vi "Scripting_ReplaceVisAndControls.vi"(0 "ViRef":refnum<vi>, 1 "OldVIsAndControls":path[](array[path]), 2 "NewVIsAndControls":path[](array[path]), 5 "error in (no error)":errorcluster) -> (15 "ReplacedVIsConPaneSize":u32[](array[numeric]), 19 "error out":errorcluster)   [LabVIEW 2020]
uses:
  <resource>/Framework/Providers/Open_GDS/ClassProviders/Common/ScriptingFunctions/Scripting.lvclass
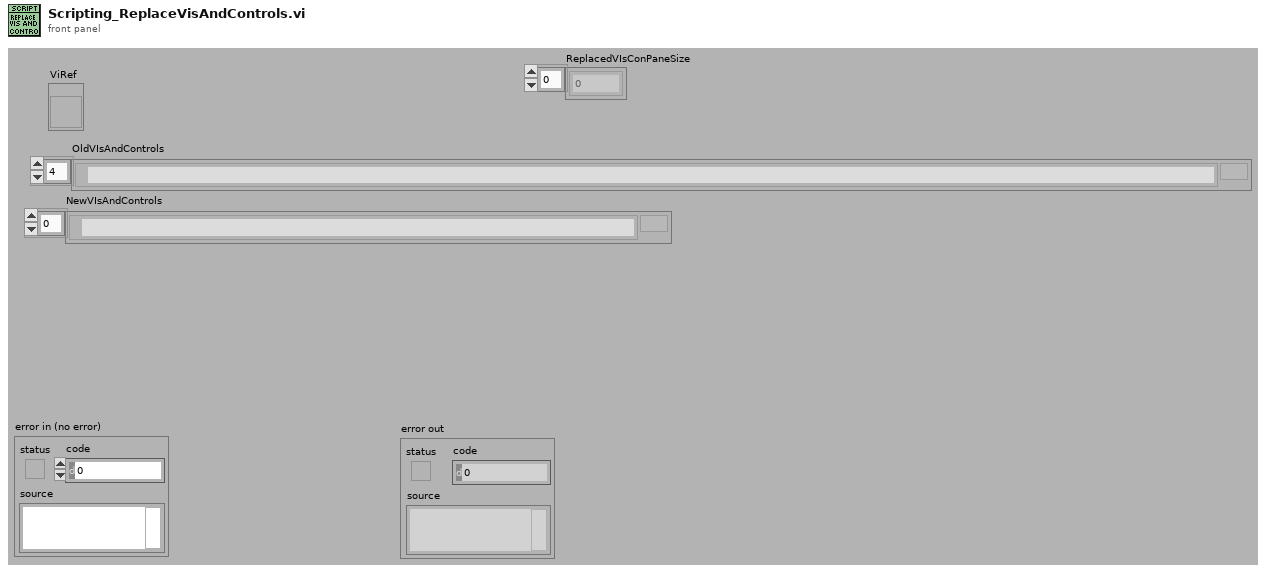
[diagram p1: front panel]
types:
  T1 = enum32{"invalid lock state", "Not Locked", "Locked (No Password)", "Password-protected"}
  T2 = cluster{"ClassControls":refnum<vi>[], "NewClassControl":path, "ReplacedVIsConPaneSize":u32[]}
  T3 = enum32{"not a typedef", "typedef", "strict typedef", "class private data"}
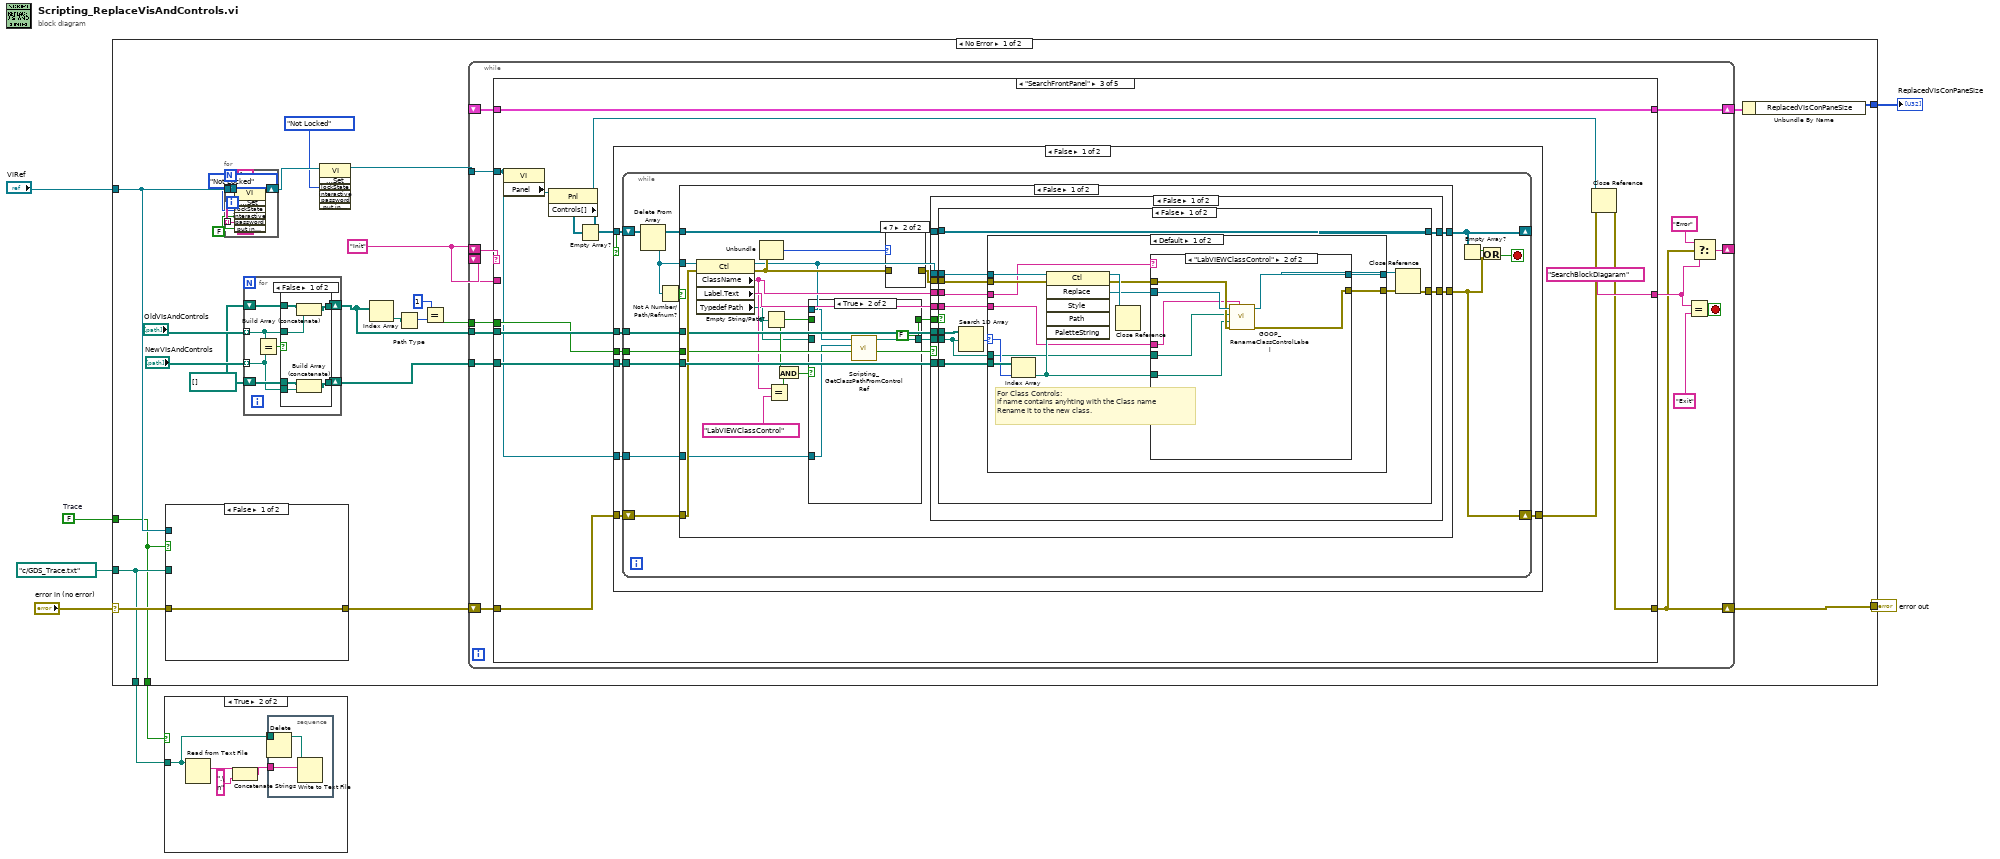
[diagram p0: block diagram]
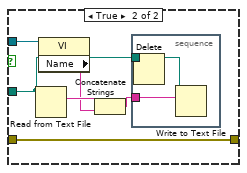
[diagram p3: hidden frame]
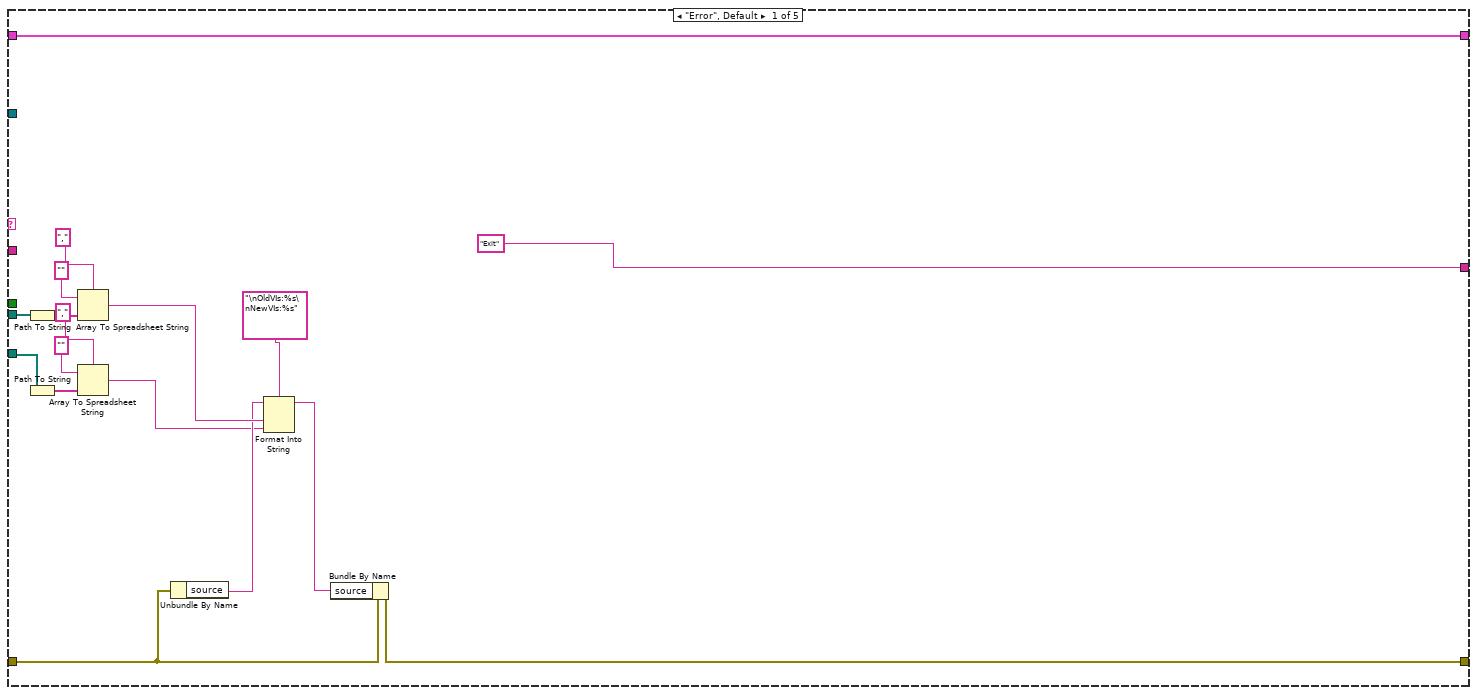
[diagram p5: hidden frame]
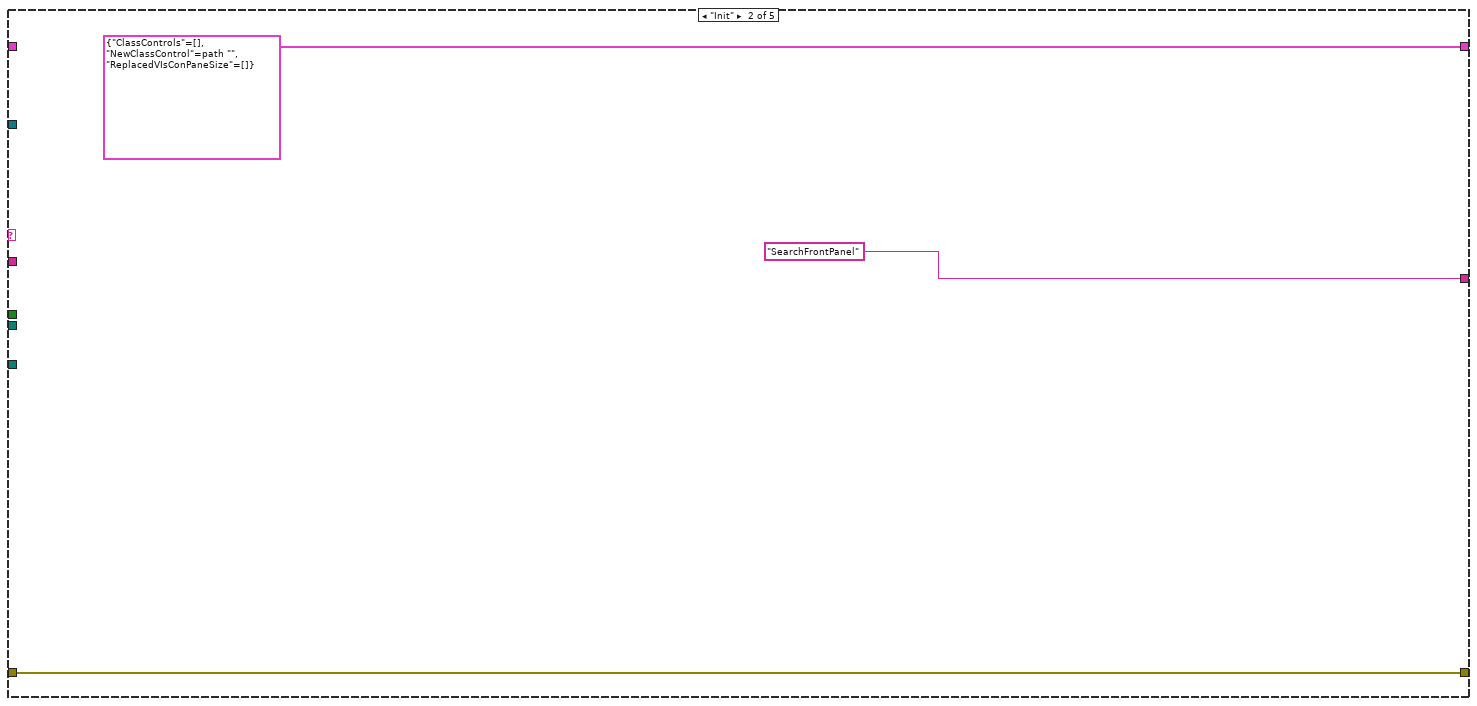
[diagram p6: hidden frame]
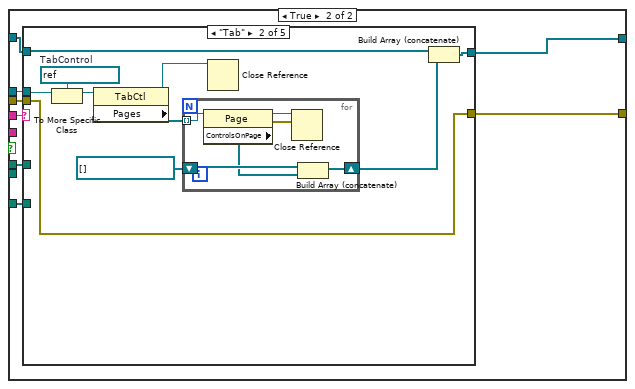
[diagram p11: hidden frame]
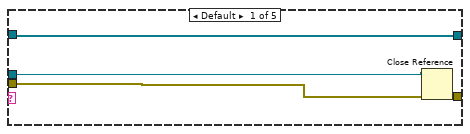
[diagram p12: hidden frame]
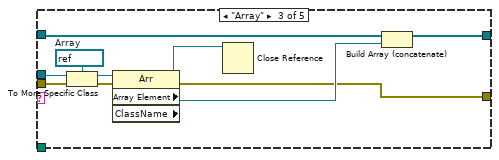
[diagram p13: hidden frame]
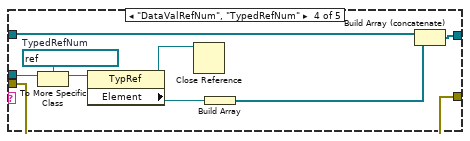
[diagram p14: hidden frame]
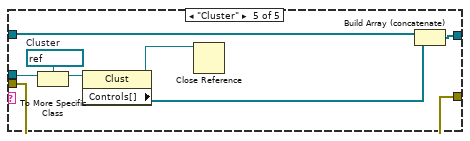
[diagram p15: hidden frame]
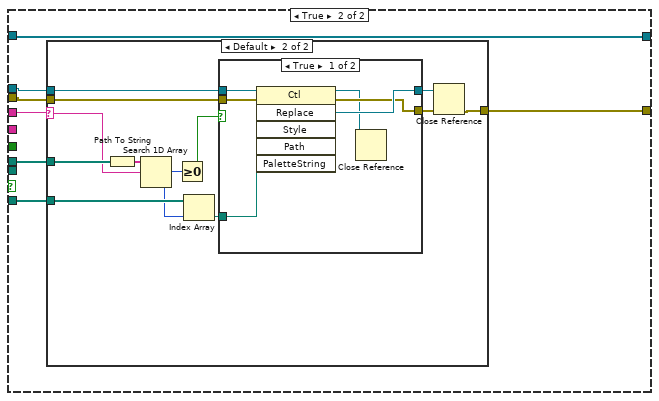
[diagram p16: hidden frame]
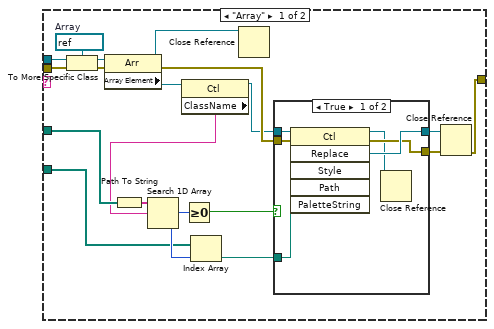
[diagram p17: hidden frame]
diagram:
  w6 = FALSE  # Trace
  n1 = case shown="No Error" "error in (no error)" {
    selector: "error in (no error)" -> [w22 w842]
    tunnel: [w30 w842] -> w8
    tunnel: "ViRef" -> [w20 _]
    tunnel: w6 -> [w18 _]
    tunnel: path "c:/GDS_Trace.txt" -> [w19 _]
    tunnel: [w19 _] -> w4
    tunnel: [w18 _] -> w3
    tunnel: [w10 _] -> w1
    frame No Error {
      w23 = path[] []
      w9 = "Init"
      n2 = case shown="False" w18 {
        tunnel: w22 -> [w31 w36]
        tunnel: [w31 w36] -> w21
        tunnel: w20 -> [_ w37]
        tunnel: w19 -> [_ w32]
        frame False {
        }
        frame True {
          n3 = Read from Text File(file (use dialog)=w32) -> (text=w35:string)  [unwired: 3 in, 3 out]
          n4 = property class="VI"(reference=w37) -> ("Name"=w34:string)  [unwired: 1 in, 2 out]
          n5 = Concatenate Strings(w35, w34) -> (w33:string)
          n6 = stacked-sequence {
            tunnel: w33 -> [w40]
            tunnel: w32 -> [w39]
            frame #0 {
              n7 = Delete(path (use dialog)=w39) -> (deleted path=w38:path)  [unwired: 4 in, 2 out]
              n8 = Write to Text File(file (use dialog)=w38, text=w40) -> ()  [unwired: 2 in, 3 out]
            }
          }
        }
      }
      n9 = for {
        tunnel: string[] ["goop rules", "i love goteborg", "Endevo Knows Goop!", "kiss"] -> [w58] mode=indexing
        shift-right: [w56] -> w28
        shift-left: w20 -> [_]
        tunnel: w20 -> [w57]
        w59 = FALSE ("Interactive")
        n10 = invoke class="VI" method="Lock State.Set"(reference=w57, "lockState"=T1."Not Locked" ("Lock State"), "interactive"=w59, "password"=w58, "put in Cache"=w59) -> (reference out=w56:refnum<vi>)  [unwired: 2 in, 6 out]
      }
      n11 = for {
        tunnel: "NewVIsAndControls" -> [w41] mode=indexing
        tunnel: "OldVIsAndControls" -> [w44] mode=indexing
        shift-right: [w45] -> w17
        shift-left: w23 -> [w46]
        shift-right: [w43] -> w13
        shift-left: w23 -> [w42]
        n12 = Equal?(x=w44, y=w41) -> (x = y?=w47:bool)
        n13 = case shown="False" w47 {
          tunnel: w46 -> [w53 w55]
          tunnel: [w52 w55] -> w45
          tunnel: w44 -> [w51 _]
          tunnel: w42 -> [w49 w54]
          tunnel: [w50 w54] -> w43
          tunnel: w41 -> [w48 _]
          frame False {
            n14 = Build Array (concatenate)(w53, w51) -> (w52:path[])
            n15 = Build Array (concatenate)(w49, w48) -> (w50:path[])
          }
          frame True {
          }
        }
      }
      n16 = invoke class="VI" method="Lock State.Set"(reference=w28, "lockState"=T1."Not Locked" ("Lock State")) -> (reference out=w26:refnum<vi>)  [unwired: 5 in, 6 out]
      n17 = Index Array(array=w17) -> (element=w14:path)  [unwired: 1 in]
      n18 = Path Type(1:w14) -> (0:w16:i16)
      n19 = Equal?(x=i16 1, y=w16) -> (x = y?=w12:bool)
      n20 = while {
        shift-right: [w68] -> w30
        shift-left: w21 -> [w75]
        shift-right: [w73] -> _
        shift-left: w9 -> [w74]
        shift-right: [w67] -> w11
        shift-left: _ -> [w66]
        tunnel: w26 -> [w63]
        tunnel: w17 -> [w65]
        tunnel: w13 -> [w64]
        tunnel: w12 -> [w62]
        shift-left: w9 -> [w61]
        stop <- w72 stop-if-true
        n21 = case shown="\"SearchFrontPanel\"" w74 {
          tunnel: w75 -> [w90 w95 w102 w324 w827]
          tunnel: [w89 w95 w101 w325 w826] -> w68
          tunnel: ["Exit" "SearchFrontPanel" "SearchBlockDiagaram" "Save" "Exit"] -> w69
          tunnel: [w91 T2 {"ClassControls"=[], "NewClassControl"=path "", "ReplacedVIsConPaneSize"=[]} w105 w318 w823] -> w67
          tunnel: w66 -> [w91 _ w105 w319 w823]
          tunnel: w63 -> [_ _ w96 w328 w828]
          tunnel: w65 -> [w88 _ w107 w323 _]
          tunnel: w64 -> [w78 _ w106 w322 _]
          tunnel: w62 -> [_ _ w97 w320 _]
          tunnel: w61 -> [_ _ _ _ _]
          frame "Error", Default {
            n22 = Path To String(path=w88) -> (string=w87:string[])
            n23 = Path To String(path=w78) -> (string=w79:string[])
            n24 = Array To Spreadsheet String(delimiter (Tab)=",", array=w87, 3:"" ("format string")) -> (spreadsheet string=w84:string)
            n25 = Array To Spreadsheet String(delimiter (Tab)=",", array=w79, 3:"" ("format string")) -> (spreadsheet string=w76:string)
            n26 = Unbundle By Name(w90) -> ("source"=w77:string)
            n27 = Format Into String(format string="\nOldVIs:%s\nNewVIs:%s", initial string=w77, w84, w76) -> (resulting string=w82:string)  [unwired: 1 in, 1 out]
            n28 = Bundle By Name(cluster=w90, "source"=w82) -> (w89:errorcluster)
          }
          frame "Init" {
          }
          frame "SearchFrontPanel" {
            n29 = property class="VI"(reference=w96) -> ("Panel"=w108:refnum<vi>)  [unwired: 1 in, 2 out]
            n30 = property class="Pnl"(reference=w108) -> (reference out=w100:refnum<vi>, "Controls[]"=w99:refnum<vi>[])  [unwired: 1 in, 1 out]
            n31 = Empty Array?(array=w99) -> (empty?=w98:bool)
            n32 = case shown="False" w98 {
              tunnel: w107 -> [w115 _]
              tunnel: w106 -> [w114 _]
              tunnel: [w113 w316] -> w103
              tunnel: w102 -> [w112 w316]
              tunnel: w99 -> [w111 _]
              tunnel: w97 -> [w110 _]
              tunnel: w96 -> [w109 _]
              frame False {
                n33 = while {
                  shift-right: [w120] -> _
                  shift-left: w111 -> [w128]
                  tunnel: w115 -> [w124]
                  tunnel: w114 -> [w126]
                  shift-right: [w117] -> w113
                  shift-left: w112 -> [w125]
                  tunnel: w110 -> [w121]
                  tunnel: w109 -> [w116]
                  stop <- w118 stop-if-true
                  n34 = Delete From Array(array=w128) -> (deleted portion=w123:refnum<vi>, array with subset deleted=w127:refnum<vi>[])  [unwired: 2 in]
                  n35 = Not A Number/Path/Refnum?(number/path/refnum=w123) -> (NaN/Path/Refnum?=w122:bool)
                  n36 = case shown="False" w122 {
                    tunnel: w127 -> [w150 w314]
                    tunnel: [w149 w314] -> w120
                    tunnel: w126 -> [w148 _]
                    tunnel: w125 -> [w147 w315]
                    tunnel: [w146 w315] -> w117
                    tunnel: w124 -> [w145 _]
                    tunnel: w123 -> [w144 _]
                    tunnel: w121 -> [w143 _]
                    tunnel: w116 -> [w129 _]
                    frame False {
                      n37 = property class="Ctl"(reference=w144, error in=w147) -> (reference out=w130:refnum<vi>, error out=w140:errorcluster, "ClassName"=w138:string, "Label.Text"=w142:string, "Typedef Path"=w131:path)
                      n38 = Unbundle(w140) -> ("code"=w141:i32)  [unwired: 2 out]
                      n39 = Empty String/Path?(string/path=w131) -> (empty?=w134:bool)
                      n40 = Equal?(x=w138, y="LabVIEWClassControl") -> (x = y?=w136:bool)
                      n41 = And(x=w134, y=w136) -> (x .and. y?=w135:bool)
                      n42 = case shown="True" w135 {
                        tunnel: w134 -> [w152 _]
                        tunnel: [w152 FALSE] -> w133
                        tunnel: w131 -> [w151 _]
                        tunnel: [w151 w156] -> w132
                        tunnel: w130 -> [_ w155]
                        tunnel: w129 -> [_ w153]
                        frame False {
                        }
                        frame True {
                          n43 = call <resource>:"Scripting_GetClassPathFromControlRef.vi"("ViRef"=w153, "Control in"=w155) -> ("class path"=w156:path)  [unwired: 9 in]
                        }
                      }
                      n44 = case shown="7" w141 {
                        tunnel: w140 -> [w157 _]
                        tunnel: [w157 _] -> w139
                        frame 0, Default {
                        }
                        frame 7 {
                        }
                      }
                      n45 = case shown="False" w143 {
                        tunnel: w138 -> [w168 w260]
                        tunnel: w130 -> [w167 w265]
                        tunnel: w150 -> [w166 w262]
                        tunnel: [w165 w262] -> w149
                        tunnel: w148 -> [w164 w263]
                        tunnel: w139 -> [w163 w264]
                        tunnel: [w162 w266] -> w146
                        tunnel: w145 -> [w161 w261]
                        tunnel: w132 -> [w160 _]
                        tunnel: w133 -> [w159 _]
                        tunnel: w142 -> [w158 _]
                        frame False {
                          n46 = case shown="False" w159 {
                            tunnel: w168 -> [w171 w212]
                            tunnel: w167 -> [w176 w211]
                            tunnel: w166 -> [w174 w210]
                            tunnel: [w174 w209] -> w165
                            tunnel: w164 -> [w177 w208]
                            tunnel: w163 -> [w175 w207]
                            tunnel: [w178 w206] -> w162
                            tunnel: w161 -> [w173 w205]
                            tunnel: w160 -> [w169 _]
                            tunnel: w158 -> [w170 _]
                            frame False {
                              n47 = Search 1D Array(1D array=w173, element=w169) -> (index of element=w172:i32)  [unwired: 1 in]
                              n48 = case shown="Default" w172 {
                                selector: w172 -> [w190 _]
                                tunnel: [w186 w204] -> w180
                                tunnel: [w184 w203] -> w179
                                tunnel: w177 -> [w192 _]
                                tunnel: w176 -> [w189 w204]
                                tunnel: w175 -> [w191 w203]
                                tunnel: w171 -> [w188 _]
                                tunnel: w170 -> [w181 _]
                                tunnel: w169 -> [w182 _]
                                frame Default {
                                # "For Class Controls:\nIf name contains anyhting with the Class name\nRename it to the new class."
                                n49 = Index Array(array=w192, index=w190) -> (element=w183:path)
                                n50 = invoke class="Ctl" method="Replace"(reference=w189, error in=w191, "Path"=w183) -> (reference out=w193:refnum<vi>, error out=w185:errorcluster, "Replace"=w187:refnum<vi>)  [unwired: 3 in, 3 out]
                                n51 = Close Reference(reference=w193) -> ()  [unwired: 1 in, 1 out]
                                n52 = case shown="\"LabVIEWClassControl\"" w188 {
                                tunnel: w187 -> [w195 w202]
                                tunnel: [w195 w201] -> w186
                                tunnel: w185 -> [w194 w199]
                                tunnel: [w194 w200] -> w184
                                tunnel: w183 -> [_ w198]
                                tunnel: w182 -> [_ w197]
                                tunnel: w181 -> [_ w196]
                                frame Default {
                                }
                                frame "LabVIEWClassControl" {
                                n53 = call <resource>:"GOOP_RenameClassControlLabel.vi"("Label.Text"=w196, "error in (no error)"=w199, "Path"=w198, "Typedef Path"=w197, "GObject in"=w202) -> ("error out"=w200:errorcluster, "Control out"=w201:refnum<vi>)  [unwired: 5 in]
                                }
                                }
                                }
                                frame -1 {
                                }
                              }
                              n54 = Close Reference(reference=w180, error in (no error)=w179) -> (error out=w178:errorcluster)
                            }
                            frame True {
                              n55 = case shown="\"Tab\"" w212 {
                                tunnel: w211 -> [w214 w226 w242 w251 w259]
                                tunnel: w210 -> [w216 w221 w236 w248 w256]
                                tunnel: [w216 w219 w233 w247 w255] -> w209
                                tunnel: w208 -> [_ _ _ _ _]
                                tunnel: w207 -> [w213 w217 w237 w245 w253]
                                tunnel: [w215 w217 w234 w245 w253] -> w206
                                tunnel: w205 -> [_ _ _ _ _]
                                frame Default {
                                n56 = Close Reference(reference=w214, error in (no error)=w213) -> (error out=w215:errorcluster)
                                }
                                frame "Tab" {
                                w225 = refnum<vi> refnum  # TabControl
                                n57 = To More Specific Class(target class=w225, reference=w226) -> (specific class reference=w224:refnum<vi>)  [unwired: 1 in, 1 out]
                                n58 = property class="TabCtl"(reference=w224) -> (reference out=w218:refnum<vi>, "Pages"=w223:refnum<vi>[])  [unwired: 1 in, 1 out]
                                n59 = for {
                                tunnel: w223 -> [w232] mode=indexing
                                shift-right: [w231] -> w220
                                shift-left: refnum<vi>[] [] -> [w230]
                                n60 = property class="Page"(reference=w232) -> (reference out=w227:refnum<vi>, error out=w228:errorcluster, "ControlsOnPage"=w229:refnum<vi>[])  [unwired: 1 in]
                                n61 = Close Reference(reference=w227, error in (no error)=w228) -> ()  [unwired: 1 out]
                                n62 = Build Array (concatenate)(w230, w229) -> (w231:refnum<vi>[])
                                }
                                n63 = Close Reference(reference=w218) -> ()  [unwired: 1 in, 1 out]
                                n64 = Build Array (concatenate)(w221, w220) -> (w219:refnum<vi>[])
                                }
                                frame "Array" {
                                w241 = refnum<vi> refnum  # Array
                                n65 = To More Specific Class(target class=w241, reference=w242, error in=w237) -> (specific class reference=w240:refnum<vi>, error out=w238:errorcluster)
                                n66 = property class="Arr" props=["Array Element", "ClassName"](reference=w240, error in=w238) -> (reference out=w239:refnum<vi>, error out=w234:errorcluster, "Array Element"=w235:refnum<vi>)  [unwired: 1 out]
                                n67 = Close Reference(reference=w239) -> ()  [unwired: 1 in, 1 out]
                                n68 = Build Array (concatenate)(w236, w235) -> (w233:refnum<vi>[])
                                }
                                frame "DataValRefNum", "TypedRefNum" {
                                w250 = refnum<vi> refnum  # TypedRefNum
                                n69 = To More Specific Class(target class=w250, reference=w251) -> (specific class reference=w249:refnum<vi>)  [unwired: 1 in, 1 out]
                                n70 = property class="TypRef"(reference=w249) -> (reference out=w246:refnum<vi>, "Element"=w244:refnum<vi>)  [unwired: 1 in, 1 out]
                                n71 = Close Reference(reference=w246) -> ()  [unwired: 1 in, 1 out]
                                n72 = Build Array(w244) -> (w243:refnum<vi>[])
                                n73 = Build Array (concatenate)(w248, w243) -> (w247:refnum<vi>[])
                                }
                                frame "Cluster" {
                                w258 = refnum<vi> refnum  # Cluster
                                n74 = To More Specific Class(target class=w258, reference=w259) -> (specific class reference=w257:refnum<vi>)  [unwired: 1 in, 1 out]
                                n75 = property class="Clust"(reference=w257) -> (reference out=w254:refnum<vi>, "Controls[]"=w252:refnum<vi>[])  [unwired: 1 in, 1 out]
                                n76 = Close Reference(reference=w254) -> ()  [unwired: 1 in, 1 out]
                                n77 = Build Array (concatenate)(w256, w252) -> (w255:refnum<vi>[])
                                }
                              }
                            }
                          }
                        }
                        frame True {
                          n78 = case shown="Default" w260 {
                            selector: w260 -> [_ w294]
                            tunnel: [w270 w303] -> w266
                            tunnel: w265 -> [w273 w302]
                            tunnel: w264 -> [w274 w301]
                            tunnel: w263 -> [w272 w300]
                            tunnel: w261 -> [w271 w298]
                            frame "Array" {
                              w285 = refnum<vi> refnum  # Array
                              n79 = To More Specific Class(target class=w285, reference=w273, error in=w274) -> (specific class reference=w284:refnum<vi>, error out=w275:errorcluster)
                              n80 = property class="Arr"(reference=w284, error in=w275) -> (reference out=w283:refnum<vi>, error out=w276:errorcluster, "Array Element"=w269:refnum<vi>)
                              n81 = Path To String(path=w271) -> (string=w279:string[])
                              n82 = property class="Ctl"(reference=w269) -> (reference out=w268:refnum<vi>, "ClassName"=w267:string)  [unwired: 1 in, 1 out]
                              n83 = Search 1D Array(1D array=w279, element=w267) -> (index of element=w277:i32)  [unwired: 1 in]
                              n84 = Greater Or Equal To 0?(x=w277) -> (x >= 0?=w278:bool)
                              n85 = Index Array(array=w272, index=w277) -> (element=w280:path)
                              n86 = Close Reference(reference=w283) -> ()  [unwired: 1 in, 1 out]
                              n87 = case shown="True" w278 {
                                tunnel: [w291 w293] -> w282
                                tunnel: [w290 w292] -> w281
                                tunnel: w268 -> [w288 w293]
                                tunnel: w276 -> [w287 w292]
                                tunnel: w280 -> [w286 _]
                                frame True {
                                n88 = invoke class="Ctl" method="Replace"(reference=w288, error in=w287, "Path"=w286) -> (reference out=w289:refnum<vi>, error out=w290:errorcluster, "Replace"=w291:refnum<vi>)  [unwired: 3 in, 3 out]
                                n89 = Close Reference(reference=w289) -> ()  [unwired: 1 in, 1 out]
                                }
                                frame False {
                                }
                              }
                              n90 = Close Reference(reference=w282, error in (no error)=w281) -> (error out=w270:errorcluster)
                            }
                            frame Default {
                              n91 = Path To String(path=w298) -> (string=w297:string[])
                              n92 = Search 1D Array(1D array=w297, element=w294) -> (index of element=w295:i32)  [unwired: 1 in]
                              n93 = Greater Or Equal To 0?(x=w295) -> (x >= 0?=w296:bool)
                              n94 = Index Array(array=w300, index=w295) -> (element=w299:path)
                              n95 = case shown="True" w296 {
                                tunnel: [w311 w313] -> w305
                                tunnel: [w310 w312] -> w304
                                tunnel: w302 -> [w308 w313]
                                tunnel: w301 -> [w307 w312]
                                tunnel: w299 -> [w306 _]
                                frame True {
                                n96 = invoke class="Ctl" method="Replace"(reference=w308, error in=w307, "Path"=w306) -> (reference out=w309:refnum<vi>, error out=w310:errorcluster, "Replace"=w311:refnum<vi>)  [unwired: 3 in, 3 out]
                                n97 = Close Reference(reference=w309) -> ()  [unwired: 1 in, 1 out]
                                }
                                frame False {
                                }
                              }
                              n98 = Close Reference(reference=w305, error in (no error)=w304) -> (error out=w303:errorcluster)
                            }
                          }
                        }
                      }
                    }
                    frame True {
                    }
                  }
                  n99 = Empty Array?(array=w120) -> (empty?=w119:bool)
                  n100 = Or(x=w119, y=w117) -> (x .or. y?=w118:bool)
                }
              }
              frame True {
              }
            }
            n101 = Close Reference(reference=w100, error in (no error)=w103) -> (error out=w101:errorcluster)
          }
          frame "SearchBlockDiagaram" {
            n102 = property class="VI"(reference=w328) -> (error out=w321:errorcluster, "Diagram"=w327:refnum<vi>)  [unwired: 1 in, 1 out]
            n103 = case shown="No Error" w321 {
              tunnel: w327 -> [w338 w821]
              tunnel: [w336 w822] -> w325
              tunnel: w324 -> [w335 w822]
              tunnel: w323 -> [w334 _]
              tunnel: w322 -> [w333 _]
              tunnel: w320 -> [w331 _]
              tunnel: [w329 _] -> w317
              frame No Error {
                n104 = property class="TopLvlDiag"(reference=w338) -> (reference out=w332:refnum<vi>, "AllObjs[]"=w337:refnum<vi>[])  [unwired: 1 in, 1 out]
                n105 = while {
                  shift-right: [w351] -> _
                  shift-left: w337 -> [w355]
                  shift-right: [w340] -> w336
                  shift-left: w335 -> [w349]
                  tunnel: w334 -> [w348]
                  tunnel: w333 -> [w347]
                  tunnel: w331 -> [w344]
                  shift-right: [w342] -> w329
                  shift-left: u32[] [] -> [w343]
                  stop <- w353 stop-if-true
                  # "LabVIEWClassConstant"
                  n106 = Delete From Array(array=w355) -> (deleted portion=w346:refnum<vi>, array with subset deleted=w352:refnum<vi>[])  [unwired: 2 in]
                  n107 = Not A Number/Path/Refnum?(number/path/refnum=w346) -> (NaN/Path/Refnum?=w345:bool)
                  n108 = case shown="False" w345 {
                    tunnel: [w369 _] -> w350
                    tunnel: [w366 w820] -> w341
                    tunnel: w349 -> [w365 w820]
                    tunnel: w348 -> [w364 _]
                    tunnel: w347 -> [w363 _]
                    tunnel: w346 -> [w362 _]
                    tunnel: w344 -> [w361 _]
                    tunnel: w343 -> [w360 w819]
                    tunnel: [w359 w819] -> w342
                    frame False {
                      n109 = property class="GObj"(reference=w362, error in=w365) -> (reference out=w371:refnum<vi>, error out=w372:errorcluster, "Class Name"=w370:string)
                      n110 = case shown="False" w361 {
                        tunnel: w372 -> [w382 w769]
                        tunnel: w371 -> [w381 w772]
                        tunnel: w370 -> [w380 w766]
                        tunnel: [w379 _] -> w369
                        tunnel: [w378 w770] -> w368
                        tunnel: [w377 w771] -> w367
                        tunnel: w364 -> [w376 w767]
                        tunnel: w363 -> [w375 w773]
                        tunnel: w360 -> [w374 w765]
                        tunnel: [w373 w765] -> w359
                        frame False {
                          n111 = case shown="Default" w380 {
                            selector: w380 -> [w392 _ _ _ _ _ _ _ _ _ _]
                            tunnel: w381 -> [w390 w603 w623 w643 w663 w683 w703 w722 w741 w752 w764]
                            tunnel: w382 -> [w391 w598 w618 w638 w660 w680 w700 w721 w737 w748 w760]
                            tunnel: [w385 w596 w616 w636 w653 w674 w696 w714 w733 w744 w755] -> w378
                            tunnel: [w386 w594 w614 w634 w655 w675 w694 w713 w735 w746 w758] -> w379
                            tunnel: [w387 w597 w617 w637 w654 w673 w695 w715 w734 w745 w757] -> w377
                            tunnel: w376 -> [w389 _ _ _ _ _ _ _ _ _ _]
                            tunnel: w375 -> [w388 _ _ _ _ _ _ _ _ _ _]
                            tunnel: w374 -> [w384 w592 w612 w632 w652 w672 w692 w712 w731 w742 w753]
                            tunnel: [w383 w592 w612 w632 w652 w672 w692 w712 w731 w742 w753] -> w373
                            frame Default {
                              n112 = case shown="Default" w392 {
                                selector: w392 -> [w394 _ _ _ _]
                                tunnel: w391 -> [w397 w481 w517 w536 w569]
                                tunnel: w390 -> [w399 w482 w518 w546 w578]
                                tunnel: [w401 w480 w516 w545 w577] -> w385
                                tunnel: [w398 w479 w515 w544 w576] -> w387
                                tunnel: w389 -> [w396 w473 w509 w540 w572]
                                tunnel: w388 -> [w395 w470 w506 w537 w570]
                                tunnel: [_ _ _ w529 w561] -> w386
                                tunnel: w384 -> [w393 w469 w505 w528 w560]
                                tunnel: [w393 w468 w505 w528 w560] -> w383
                                frame Default {
                                w403 = refnum<vi> refnum  # Constant
                                n113 = To More Specific Class(target class=w403, reference=w399, error in=w397) -> (specific class reference=w402:refnum<vi>, error out=w400:errorcluster)
                                n114 = case shown="No Error" w400 {
                                selector: w400 -> [w413 _]
                                tunnel: w402 -> [w409 _]
                                tunnel: [w414 w466] -> w401
                                tunnel: w399 -> [w407 w467]
                                tunnel: [w412 w467] -> w398
                                tunnel: w397 -> [w408 w466]
                                tunnel: w396 -> [w406 _]
                                tunnel: w395 -> [w404 _]
                                tunnel: w394 -> [w410 _]
                                frame No Error {
                                n115 = case shown="\"LabVIEWClassConstant\"" w410 {
                                tunnel: w409 -> [_ w461]
                                tunnel: w413 -> [w433 w460]
                                tunnel: [w426 w459] -> w411
                                tunnel: w407 -> [w434 _]
                                tunnel: w406 -> [w432 w458]
                                tunnel: [w427 w457] -> w405
                                frame "LabVIEWClassConstant" {
                                w435 = refnum<vi> refnum  # LabVIEWClassConstant
                                n116 = for {
                                tunnel: w432 -> [w454] mode=indexing
                                tunnel: [w453] -> w431 mode=indexing
                                n117 = Strip Path(path=w454) -> (name=w453:string)  [unwired: 1 out]
                                }
                                n118 = To More Specific Class(target class=w435, reference=w434, error in=w433) -> (specific class reference=w437:refnum<vi>, error out=w436:errorcluster)
                                n119 = disable-structure shown="Enabled" {
                                disable-tunnel: w437 -> [w444 _]
                                disable-tunnel: w436 -> [w443 w452]
                                disable-tunnel: [w442 "-1"] -> w428
                                disable-tunnel: [w438 w452] -> w426
                                frame Enabled {
                                n120 = property class="LVClassConstant"(reference=w444, error in=w443) -> (error out=w438:errorcluster, "Value"=w445:variant)  [unwired: 1 out]
                                n121 = Flatten To String(anything=w445) -> (data string=w446:string)  [unwired: 3 in, 2 out]
                                n122 = Match Pattern(string=w446, regular expression="[~\\00\\01\\02\\03\\04\\05\\06\\07\\08\\09\\0A\\0B\\0C\\0D\\0E\\0F\\10\\11\\12\\13\\14\\15\\16\\17\\18\\19\\1A\\1B\\1C\\1D\\1E]+\\.lvclass") -> (match substring=w440:string)  [unwired: 1 in, 3 out]
                                n123 = Match Pattern(string=w440, regular expression="[~A-Za-zäöåÄÖÅÜü_]*") -> (after substring=w439:string)  [unwired: 1 in, 3 out]
                                n124 = Match Pattern(string=w439, regular expression="\\.lvclass") -> (before substring=w450:string)  [unwired: 1 in, 3 out]
                                n125 = Format Into String(format string="%s.ctl", w450) -> (resulting string=w442:string)  [unwired: 2 in, 1 out]
                                }
                                frame Disabled {
                                }
                                }
                                n126 = To Lower Case(string=w431) -> (all lower case string=w430:string[])
                                n127 = To Lower Case(string=w428) -> (all lower case string=w429:string)
                                n128 = Search 1D Array(1D array=w430, element=w429) -> (index of element=w427:i32)  [unwired: 1 in]
                                }
                                frame Default {
                                n129 = property class="Const"(reference=w461, error in=w460) -> (error out=w459:errorcluster, "Typedef Path"=w456:path)  [unwired: 1 out]
                                n130 = Empty String/Path?(string/path=w456) -> (empty?=w455:bool)
                                n131 = case shown="False" w455 {
                                tunnel: w458 -> [w464 _]
                                tunnel: [w463 -1 ("index of element")] -> w457
                                tunnel: w456 -> [w462 _]
                                frame False {
                                n132 = Search 1D Array(1D array=w464, element=w462) -> (index of element=w463:i32)  [unwired: 1 in]
                                }
                                frame True {
                                }
                                }
                                }
                                }
                                n133 = case shown="0, Default" w405 {
                                selector: w405 -> [w421 _]
                                tunnel: w408 -> [w422 w424]
                                tunnel: w409 -> [w423 w425]
                                tunnel: [w417 w425] -> w412
                                tunnel: [w416 w424] -> w414
                                tunnel: w404 -> [w420 _]
                                tunnel: w411 -> [_ _]
                                tunnel: [w415 _] -> _
                                frame 0, Default {
                                n134 = Index Array(array=w420, index=w421) -> (element=w419:path)
                                n135 = invoke class="Const" method="Replace"(reference=w423, error in=w422, "Path"=w419) -> (reference out=w418:refnum<vi>, error out=w416:errorcluster, "Replace"=w417:refnum<vi>)  [unwired: 3 in, 3 out]
                                n136 = Close Reference(reference=w418) -> (error out=w415:errorcluster)  [unwired: 1 in]
                                }
                                frame -1 {
                                }
                                }
                                }
                                frame Error {
                                }
                                }
                                }
                                frame "PolymorphicSubVI", "SubVI" {
                                n137 = To More Specific Class(target class=refnum<vi> refnum ("WhileLoop"), reference=w482, error in=w481) -> (specific class reference=w477:refnum<vi>, error out=w476:errorcluster)
                                n138 = property class="SubVI"(reference=w477, error in=w476) -> (reference out=w474:refnum<vi>, error out=w475:errorcluster, "VI Path"=w472:path)
                                n139 = Search 1D Array(1D array=w473, element=w472) -> (index of element=w471:i32)  [unwired: 1 in]
                                n140 = case shown="0, Default" w471 {
                                selector: w471 -> [w501 _]
                                tunnel: w475 -> [w498 w503]
                                tunnel: w474 -> [w499 w504]
                                tunnel: [w494 w504] -> w479
                                tunnel: [w493 w503] -> w480
                                tunnel: w470 -> [w500 _]
                                tunnel: [w487 _] -> _
                                tunnel: w469 -> [w485 w502]
                                tunnel: [w483 w502] -> w468
                                frame 0, Default {
                                n141 = Index Array(array=w500, index=w501) -> (element=w497:path)
                                n142 = call <resource>:"Scripting_ReplaceSubVI.vi"("error in"=w498, "NewVIToReplaceWith"=w497, "CurrentSubVI"=w499) -> ("error out"=w493:errorcluster, "ReplacedObject(SubVI)"=w494:refnum<vi>)  [unwired: 7 in]
                                n143 = To More Specific Class(target class=refnum<vi> refnum ("WhileLoop"), reference=w494, error in=w493) -> (specific class reference=w492:refnum<vi>, error out=w491:errorcluster)
                                n144 = property class="SubVI"(reference=w492, error in=w491) -> ("VI Ref"=w490:refnum<vi>)  [unwired: 2 out]
                                n145 = property class="VI" props=["Exec.State", "ConPane"](reference=w490) -> (reference out=w486:refnum<vi>, "ConPane"=w496:refnum<vi>)  [unwired: 1 in, 2 out]
                                n146 = property class="ConPane"(reference=w496) -> (reference out=w488:refnum<vi>, error out=w489:errorcluster, "NumConns"=w484:u32)  [unwired: 1 in]
                                n147 = Build Array (concatenate)(w485, w484) -> (w483:u32[])
                                n148 = Close Reference(reference=w488, error in (no error)=w489) -> (error out=w487:errorcluster)
                                n149 = Close Reference(reference=w486, error in (no error)=w487) -> ()  [unwired: 1 out]
                                }
                                frame -1 {
                                }
                                }
                                }
                                frame "StaticVIReference" {
                                n150 = To More Specific Class(target class=refnum<vi> refnum ("WhileLoop"), reference=w518, error in=w517) -> (specific class reference=w513:refnum<vi>, error out=w512:errorcluster)
                                n151 = property class="StatVIRef"(reference=w513, error in=w512) -> (reference out=w510:refnum<vi>, error out=w511:errorcluster, "Path"=w508:path)
                                n152 = Search 1D Array(1D array=w509, element=w508) -> (index of element=w507:i32)  [unwired: 1 in]
                                n153 = case shown="0, Default" w507 {
                                selector: w507 -> [w525 _]
                                tunnel: w511 -> [w522 w526]
                                tunnel: w510 -> [w523 w527]
                                tunnel: [w520 w527] -> w515
                                tunnel: [w519 w526] -> w516
                                tunnel: w506 -> [w524 _]
                                frame 0, Default {
                                n154 = Index Array(array=w524, index=w525) -> (element=w521:path)
                                n155 = property class="StatVIRef"(reference=w523, error in=w522, "Path"=w521) -> (reference out=w520:refnum<vi>, error out=w519:errorcluster)
                                }
                                frame -1 {
                                }
                                }
                                }
                                frame "ClusterConstant" {
                                n156 = To More Specific Class(target class=refnum<vi> refnum ("WhileLoop"), reference=w546, error in=w536) -> (specific class reference=w542:refnum<vi>, error out=w541:errorcluster)
                                n157 = property class="ClustCnst"(reference=w542, error in=w541) -> (reference out=w534:refnum<vi>, error out=w533:errorcluster, "Typedef Path"=w539:path)
                                n158 = Search 1D Array(1D array=w540, element=w539) -> (index of element=w538:i32)  [unwired: 1 in]
                                n159 = property class="ClustCnst"(reference=w534, error in=w533) -> (reference out=w532:refnum<vi>, "Elements[]"=w530:refnum<vi>[], "Typedef?"=w535:T3)  [unwired: 1 out]
                                n160 = Not Equal To 0?(x=w535) -> (x != 0?=w531:bool)
                                n161 = case shown="True" w531 {
                                tunnel: [w547 _] -> w529
                                tunnel: w530 -> [w547 w548]
                                frame False {
                                }
                                frame True {
                                n162 = for {
                                tunnel: w548 -> [w549] mode=indexing
                                n163 = Close Reference(reference=w549) -> ()  [unwired: 1 in, 1 out]
                                }
                                }
                                }
                                n164 = case shown="0, Default" w538 {
                                selector: w538 -> [w555 _]
                                tunnel: w536 -> [w556 w558]
                                tunnel: w532 -> [w557 w559]
                                tunnel: [w551 w559] -> w544
                                tunnel: [w550 w558] -> w545
                                tunnel: w537 -> [w554 _]
                                frame 0, Default {
                                n165 = Index Array(array=w554, index=w555) -> (element=w553:path)
                                n166 = invoke class="ClustCnst" method="Replace"(reference=w557, error in=w556, "Path"=w553) -> (reference out=w552:refnum<vi>, error out=w550:errorcluster, "Replace"=w551:refnum<vi>)  [unwired: 3 in, 3 out]
                                n167 = Close Reference(reference=w552) -> ()  [unwired: 1 in, 1 out]
                                }
                                frame -1 {
                                }
                                }
                                }
                                frame "ArrayConstant" {
                                n168 = To More Specific Class(target class=refnum<vi> refnum ("WhileLoop"), reference=w578, error in=w569) -> (specific class reference=w574:refnum<vi>, error out=w573:errorcluster)
                                n169 = property class="ArrCnst"(reference=w574, error in=w573) -> (reference out=w564:refnum<vi>, error out=w565:errorcluster, "Typedef Path"=w571:path)
                                n170 = Search 1D Array(1D array=w572, element=w571) -> (index of element=w562:i32)  [unwired: 1 in]
                                n171 = property class="ArrCnst"(reference=w564, error in=w565) -> (reference out=w563:refnum<vi>, "Element"=w566:refnum<vi>, "Typedef?"=w568:T3)  [unwired: 1 out]
                                n172 = Not Equal To 0?(x=w568) -> (x != 0?=w567:bool)
                                n173 = case shown="False" w567 {
                                tunnel: w566 -> [w580 w581]
                                tunnel: [w579 _] -> w561
                                frame False {
                                n174 = Build Array(w580) -> (w579:refnum<vi>[])
                                }
                                frame True {
                                n175 = Close Reference(reference=w581) -> ()  [unwired: 1 in, 1 out]
                                }
                                }
                                n176 = case shown="0, Default" w562 {
                                selector: w562 -> [w587 _]
                                tunnel: w569 -> [w588 w590]
                                tunnel: w563 -> [w589 w591]
                                tunnel: [w583 w591] -> w576
                                tunnel: [w582 w590] -> w577
                                tunnel: w570 -> [w586 _]
                                frame 0, Default {
                                n177 = Index Array(array=w586, index=w587) -> (element=w585:path)
                                n178 = invoke class="ArrCnst" method="Replace"(reference=w589, error in=w588, "Path"=w585) -> (reference out=w584:refnum<vi>, error out=w582:errorcluster, "Replace"=w583:refnum<vi>)  [unwired: 3 in, 3 out]
                                n179 = Close Reference(reference=w584) -> ()  [unwired: 1 in, 1 out]
                                }
                                frame -1 {
                                }
                                }
                                }
                              }
                            }
                            frame "CaseSelector", "CaseStructure" {
                              n180 = To More Specific Class(target class=refnum<vi> refnum ("CaseSelector"), reference=w603, error in=w598) -> (specific class reference=w601:refnum<vi>, error out=w599:errorcluster)
                              n181 = property class="CaseSel"(reference=w601, error in=w599) -> (reference out=w597:refnum<vi>, error out=w595:errorcluster, "Frames[]"=w600:refnum<vi>[])
                              n182 = for {
                                tunnel: w600 -> [w611] mode=indexing
                                shift-right: [w604] -> w596
                                shift-left: w595 -> [w610]
                                shift-right: [w607] -> w594
                                shift-left: refnum<vi>[] [] -> [w609]
                                n183 = property class="Diag"(reference=w611, error in=w610) -> (reference out=w605:refnum<vi>, error out=w606:errorcluster, "AllObjs[]"=w608:refnum<vi>[])
                                n184 = Build Array (concatenate)(w609, w608) -> (w607:refnum<vi>[])
                                n185 = Close Reference(reference=w605, error in (no error)=w606) -> (error out=w604:errorcluster)
                              }
                            }
                            frame "InPlaceElementStructure" {
                              n186 = To More Specific Class(target class=refnum<vi> refnum ("CaseSelector"), reference=w623, error in=w618) -> (specific class reference=w621:refnum<vi>, error out=w619:errorcluster)
                              n187 = property class="InPlaceStruct"(reference=w621, error in=w619) -> (reference out=w617:refnum<vi>, error out=w615:errorcluster, "Diagrams"=w620:refnum<vi>[])
                              n188 = for {
                                tunnel: w620 -> [w631] mode=indexing
                                shift-right: [w624] -> w616
                                shift-left: w615 -> [w630]
                                shift-right: [w627] -> w614
                                shift-left: refnum<vi>[] [] -> [w629]
                                n189 = property class="Diag"(reference=w631, error in=w630) -> (reference out=w625:refnum<vi>, error out=w626:errorcluster, "AllObjs[]"=w628:refnum<vi>[])
                                n190 = Build Array (concatenate)(w629, w628) -> (w627:refnum<vi>[])
                                n191 = Close Reference(reference=w625, error in (no error)=w626) -> (error out=w624:errorcluster)
                              }
                            }
                            frame "DisableStructure" {
                              n192 = To More Specific Class(target class=refnum<vi> refnum ("CaseSelector"), reference=w643, error in=w638) -> (specific class reference=w641:refnum<vi>, error out=w639:errorcluster)
                              n193 = property class="DisableStructure"(reference=w641, error in=w639) -> (reference out=w637:refnum<vi>, error out=w635:errorcluster, "Frames[]"=w640:refnum<vi>[])
                              n194 = for {
                                tunnel: w640 -> [w651] mode=indexing
                                shift-right: [w644] -> w636
                                shift-left: w635 -> [w650]
                                shift-right: [w647] -> w634
                                shift-left: refnum<vi>[] [] -> [w649]
                                n195 = property class="Diag"(reference=w651, error in=w650) -> (reference out=w645:refnum<vi>, error out=w646:errorcluster, "AllObjs[]"=w648:refnum<vi>[])
                                n196 = Build Array (concatenate)(w649, w648) -> (w647:refnum<vi>[])
                                n197 = Close Reference(reference=w645, error in (no error)=w646) -> (error out=w644:errorcluster)
                              }
                            }
                            frame "MultiFrameStructure" {
                              (unwired) string[] []
                              n198 = To More Specific Class(target class=refnum<vi> refnum ("MultiFrameStructure"), reference=w663, error in=w660) -> (specific class reference=w662:refnum<vi>, error out=w661:errorcluster)
                              n199 = property class="MFStruct"(reference=w662, error in=w661) -> (reference out=w654:refnum<vi>, error out=w657:errorcluster, "Frames[]"=w656:refnum<vi>[])
                              n200 = for {
                                tunnel: w656 -> [w671] mode=indexing
                                shift-right: [w664] -> w653
                                shift-left: w657 -> [w670]
                                shift-right: [w667] -> w655
                                shift-left: refnum<vi>[] [] -> [w669]
                                n201 = property class="Diag"(reference=w671, error in=w670) -> (reference out=w665:refnum<vi>, error out=w666:errorcluster, "AllObjs[]"=w668:refnum<vi>[])
                                n202 = Build Array (concatenate)(w669, w668) -> (w667:refnum<vi>[])
                                n203 = Close Reference(reference=w665, error in (no error)=w666) -> (error out=w664:errorcluster)
                              }
                            }
                            frame "EventStructure" {
                              n204 = To More Specific Class(target class=refnum<vi> refnum ("EventStructure"), reference=w683, error in=w680) -> (specific class reference=w682:refnum<vi>, error out=w681:errorcluster)
                              n205 = property class="EvntStruct"(reference=w682, error in=w681) -> (reference out=w673:refnum<vi>, error out=w677:errorcluster, "Frames[]"=w676:refnum<vi>[])
                              n206 = for {
                                tunnel: w676 -> [w691] mode=indexing
                                shift-right: [w684] -> w674
                                shift-left: w677 -> [w690]
                                shift-right: [w687] -> w675
                                shift-left: refnum<vi>[] [] -> [w689]
                                n207 = property class="Diag"(reference=w691, error in=w690) -> (reference out=w685:refnum<vi>, error out=w686:errorcluster, "AllObjs[]"=w688:refnum<vi>[])
                                n208 = Build Array (concatenate)(w689, w688) -> (w687:refnum<vi>[])
                                n209 = Close Reference(reference=w685, error in (no error)=w686) -> (error out=w684:errorcluster)
                              }
                            }
                            frame "Sequence" {
                              n210 = To More Specific Class(target class=refnum<vi> refnum ("Sequence"), reference=w703, error in=w700) -> (specific class reference=w702:refnum<vi>, error out=w701:errorcluster)
                              n211 = property class="Seq"(reference=w702, error in=w701) -> (reference out=w695:refnum<vi>, error out=w697:errorcluster, "Frames[]"=w693:refnum<vi>[])
                              n212 = for {
                                tunnel: w693 -> [w711] mode=indexing
                                shift-right: [w704] -> w696
                                shift-left: w697 -> [w710]
                                shift-right: [w707] -> w694
                                shift-left: refnum<vi>[] [] -> [w709]
                                n213 = property class="Diag"(reference=w711, error in=w710) -> (reference out=w705:refnum<vi>, error out=w706:errorcluster, "AllObjs[]"=w708:refnum<vi>[])
                                n214 = Build Array (concatenate)(w709, w708) -> (w707:refnum<vi>[])
                                n215 = Close Reference(reference=w705, error in (no error)=w706) -> (error out=w704:errorcluster)
                              }
                            }
                            frame "FlatSequence" {
                              n216 = To More Specific Class(target class=refnum<vi> refnum ("FlatSequence"), reference=w722, error in=w721) -> (specific class reference=w719:refnum<vi>)  [unwired: 1 out]
                              n217 = property class="FlatSeq"(reference=w719) -> (reference out=w715:refnum<vi>, error out=w717:errorcluster, "Diagrams[]"=w716:refnum<vi>[])  [unwired: 1 in]
                              n218 = for {
                                tunnel: w716 -> [w730] mode=indexing
                                shift-right: [w723] -> w714
                                shift-left: w717 -> [w729]
                                shift-right: [w726] -> w713
                                shift-left: refnum<vi>[] [] -> [w728]
                                n219 = property class="Diag"(reference=w730, error in=w729) -> (reference out=w724:refnum<vi>, error out=w725:errorcluster, "AllObjs[]"=w727:refnum<vi>[])
                                n220 = Build Array (concatenate)(w728, w727) -> (w726:refnum<vi>[])
                                n221 = Close Reference(reference=w724, error in (no error)=w725) -> (error out=w723:errorcluster)
                              }
                            }
                            frame "WhileLoop" {
                              n222 = To More Specific Class(target class=refnum<vi> refnum ("WhileLoop"), reference=w741, error in=w737) -> (specific class reference=w740:refnum<vi>, error out=w738:errorcluster)
                              n223 = property class="WLoop"(reference=w740, error in=w738) -> (reference out=w734:refnum<vi>, error out=w733:errorcluster, "Diagram"=w736:refnum<vi>)
                              n224 = property class="Diag"(reference=w736) -> (reference out=w732:refnum<vi>, "AllObjs[]"=w735:refnum<vi>[])  [unwired: 1 in, 1 out]
                              n225 = Close Reference(reference=w732) -> ()  [unwired: 1 in, 1 out]
                            }
                            frame "TimedLoop" {
                              n226 = To More Specific Class(target class=refnum<vi> refnum ("WhileLoop"), reference=w752, error in=w748) -> (specific class reference=w751:refnum<vi>, error out=w749:errorcluster)
                              n227 = property class="WLoop"(reference=w751, error in=w749) -> (reference out=w745:refnum<vi>, error out=w744:errorcluster, "Diagram"=w747:refnum<vi>)
                              n228 = property class="Diag"(reference=w747) -> (reference out=w743:refnum<vi>, "AllObjs[]"=w746:refnum<vi>[])  [unwired: 1 in, 1 out]
                              n229 = Close Reference(reference=w743) -> ()  [unwired: 1 in, 1 out]
                            }
                            frame "ForLoop" {
                              n230 = To More Specific Class(target class=refnum<vi> refnum ("WhileLoop"), reference=w764, error in=w760) -> (specific class reference=w763:refnum<vi>, error out=w761:errorcluster)
                              n231 = property class="FLoop"(reference=w763, error in=w761) -> (reference out=w757:refnum<vi>, error out=w756:errorcluster, "Diagram"=w759:refnum<vi>)
                              n232 = property class="Diag"(reference=w759, error in=w756) -> (reference out=w754:refnum<vi>, error out=w755:errorcluster, "AllObjs[]"=w758:refnum<vi>[])
                              n233 = Close Reference(reference=w754, error in (no error)=w755) -> ()  [unwired: 1 out]
                            }
                          }
                        }
                        frame True {
                          n234 = Path To String(path=w767) -> (string=w768:string[])
                          n235 = case shown="Default" w766 {
                            selector: w766 -> [_ w801]
                            tunnel: w773 -> [w778 w810]
                            tunnel: w772 -> [w790 w809]
                            tunnel: [w784 w807] -> w771
                            tunnel: [w783 w806] -> w770
                            tunnel: w769 -> [w791 w805]
                            tunnel: w768 -> [w782 w804]
                            frame "ArrayConstant" {
                              n236 = To More Specific Class(target class=refnum<vi> refnum ("WhileLoop"), reference=w790, error in=w791) -> (specific class reference=w789:refnum<vi>, error out=w788:errorcluster)
                              n237 = property class="ArrCnst"(reference=w789, error in=w788) -> (reference out=w776:refnum<vi>, error out=w775:errorcluster, "Element"=w781:refnum<vi>)
                              n238 = property class="Const"(reference=w781, error in=w775) -> (reference out=w780:refnum<vi>, error out=w777:errorcluster, "Class Name"=w779:string)
                              n239 = Search 1D Array(1D array=w782, element=w779) -> (index of element=w785:i32)  [unwired: 1 in]
                              n240 = Close Reference(reference=w776, error in (no error)=w777) -> (error out=w774:errorcluster)
                              n241 = Greater Or Equal To 0?(x=w785) -> (x >= 0?=w786:bool)
                              n242 = Index Array(array=w778, index=w785) -> (element=w787:path)
                              n243 = case shown="True" w786 {
                                tunnel: w780 -> [w794 w800]
                                tunnel: w787 -> [_ w799]
                                tunnel: [w794 w796] -> w784
                                tunnel: [w793 w798] -> w783
                                tunnel: w774 -> [w793 w797]
                                frame False {
                                }
                                frame True {
                                n244 = invoke class="Const" method="Replace"(reference=w800, error in=w797, "Path"=w799) -> (reference out=w795:refnum<vi>, error out=w798:errorcluster, "Replace"=w796:refnum<vi>)  [unwired: 3 in, 3 out]
                                n245 = Close Reference(reference=w795) -> ()  [unwired: 1 in, 1 out]
                                }
                              }
                            }
                            frame Default {
                              n246 = Search 1D Array(1D array=w804, element=w801) -> (index of element=w802:i32)  [unwired: 1 in]
                              n247 = Greater Or Equal To 0?(x=w802) -> (x >= 0?=w803:bool)
                              n248 = Index Array(array=w810, index=w802) -> (element=w808:path)
                              n249 = case shown="True" w803 {
                                tunnel: w809 -> [w812 w818]
                                tunnel: w808 -> [_ w817]
                                tunnel: [w812 w814] -> w807
                                tunnel: [w811 w816] -> w806
                                tunnel: w805 -> [w811 w815]
                                frame False {
                                }
                                frame True {
                                n250 = invoke class="GObj" method="Replace"(reference=w818, error in=w815, "Path"=w817) -> (reference out=w813:refnum<vi>, error out=w816:errorcluster, "Replace"=w814:refnum<vi>)  [unwired: 3 in, 3 out]
                                n251 = Close Reference(reference=w813) -> ()  [unwired: 1 in, 1 out]
                                }
                              }
                            }
                          }
                        }
                      }
                      n252 = Close Reference(reference=w367, error in (no error)=w368) -> (error out=w366:errorcluster)
                    }
                    frame True {
                    }
                  }
                  n253 = Build Array (concatenate)(w352, w350) -> (w351:refnum<vi>[])
                  n254 = Array Size(array=w351) -> (size(s)=w354:i32)
                  n255 = Equal To 0?(x=w354) -> (x = 0?=w353:bool)
                  n256 = Unbundle(w341) -> ("code"=w339:i32)  [unwired: 2 out]
                  n257 = case shown="0, Default" w339 {
                    tunnel: w341 -> [w356 w358]
                    tunnel: [w356 w357] -> w340
                    frame 0, Default {
                    }
                    frame 1099 {
                      n258 = call <vilib>:"Clear Errors.vi"("error in (no error)"=w358) -> ("error out"=w357:errorcluster)  [unwired: 5 in, 1 out]
                    }
                  }
                }
                n259 = Close Reference(reference=w332) -> ()  [unwired: 1 in, 1 out]
              }
              frame Error {
                n260 = Close Reference(reference=w821) -> ()  [unwired: 1 in, 1 out]
              }
            }
            n261 = Bundle By Name(cluster=w319, "ReplacedVIsConPaneSize"=w317) -> (w318:T2)
          }
          frame "Save" {
            n262 = case shown="True" TRUE {
              tunnel: w828 -> [_ w838]
              tunnel: w827 -> [w829 w837]
              tunnel: [w829 w830] -> w826
              frame False {
              }
              frame True {
                w832 = FALSE  # IgnoreLibrarySaving
                n263 = invoke class="VI" method="Save.Instrument"(reference=w838, error in=w837) -> (reference out=w836:refnum<vi>, error out=w835:errorcluster)  [unwired: 4 in, 4 out]
                n264 = property class="VI"(reference=w836, error in=w835) -> (error out=w830:errorcluster, "Library"=w831:refnum<vi>)  [unwired: 1 out]
                n265 = Not A Number/Path/Refnum?(number/path/refnum=w831) -> (NaN/Path/Refnum?=w833:bool)
                n266 = Or(x=w833, y=w832) -> (x .or. y?=w834:bool)
                n267 = case shown="True" w834 {
                  tunnel: w831 -> [w840 w841]
                  frame False {
                    n268 = invoke class="Library" method="Save"(reference=w840) -> (reference out=w839:refnum<vi>)  [unwired: 3 in, 3 out]
                    n269 = Close Reference(reference=w839) -> ()  [unwired: 1 in, 1 out]
                  }
                  frame True {
                    n270 = Close Reference(reference=w841) -> ()  [unwired: 1 in, 1 out]
                  }
                }
              }
            }
          }
        }
        n271 = Equal?(x=w69, y="Exit") -> (x = y?=w72:bool)
        n272 = Select(t="Error", s=w68, f=w69) -> (s? t:f=w73:string)
      }
      n273 = Unbundle By Name(w11) -> ("ReplacedVIsConPaneSize"=w10:u32[])
    }
    frame Error {
    }
  }
  "error out" <- w8
  "ReplacedVIsConPaneSize" <- w1
  n274 = case shown="True" w3 {
    tunnel: w4 -> [_ w843]
    frame False {
    }
    frame True {
      n275 = Read from Text File(file (use dialog)=w843) -> (text=w846:string)  [unwired: 3 in, 3 out]
      n276 = Concatenate Strings(w846, ".\n" ("string")) -> (w844:string)
      n277 = stacked-sequence {
        tunnel: w844 -> [w849]
        tunnel: w843 -> [w848]
        frame #0 {
          n278 = Delete(path (use dialog)=w848) -> (deleted path=w847:path)  [unwired: 4 in, 2 out]
          n279 = Write to Text File(file (use dialog)=w847, text=w849) -> ()  [unwired: 2 in, 3 out]
        }
      }
    }
  }
